vi "Check If User Data File is Empty.vi"(8 "error in (no error)":errorcluster, 11 "Refnum in":T1) -> (0 "error out":errorcluster, 3 "Refnum out":T1)   [LabVIEW 2018]
uses:
  <vilib>/Utility/config.llb/Config Data RefNum.ctl
  <vilib>/Utility/config.llb/Write Key (String).vi
  <vilib>/Utility/config.llb/NI_LVConfig.lvlib
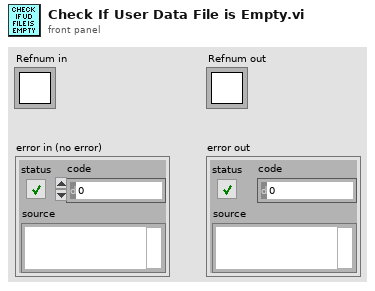
[diagram p1: front panel]
types:
  T1 = typedef "NI_LVConfig.lvlib/Config Data RefNum.ctl" = refnum<k1>
  T2 = enum16{"open", "replace", "create", "open or create", "replace or create", "replace or create with confirmation"}
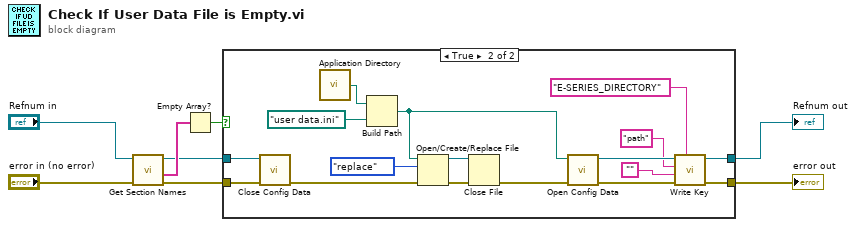
[diagram p0: block diagram]
diagram:
  n1 = call <vilib>:"Get Section Names.vi"("error in (no error)"="error in (no error)", "refnum"="Refnum in") -> ("error out"=w5:errorcluster, "section names"=w6:string[], "refnum out"=w3:T1)  [unwired: 7 in]
  n2 = Empty Array?(array=w6) -> (empty?=w4:bool)
  n3 = case shown="True" w4 {
    tunnel: w3 -> [w9 w22]
    tunnel: w5 -> [w10 w21]
    tunnel: [w10 w24] -> w8
    tunnel: [w9 w18] -> w1
    frame False {
    }
    frame True {
      n4 = call <vilib>:"Close Config Data.vi"("error in (no error)"=w21, "refnum"=w22) -> ("error out"=w17:errorcluster)  [unwired: 8 in, 1 out]
      n5 = call <vilib>:"Application Directory.vi"() -> ("Application Directory"=w20:path)
      n6 = Build Path(base path=w20, name or relative path=path "user data.ini") -> (appended path=w11:path)
      n7 = Open/Create/Replace File(file path (use dialog)=w11, error in=w17, operation (0:open)=T2."replace") -> (refnum out=w14:refnum<file>, error out=w15:errorcluster)  [unwired: 3 in, 1 out]
      n8 = Close File(refnum=w14, error in=w15) -> (error out=w13:errorcluster)  [unwired: 1 out]
      n9 = call <vilib>:"Open Config Data.vi"("error in (no error)"=w13, "configuration file path"=w11) -> ("error out"=w12:errorcluster, "refnum"=w27:T1)  [unwired: 7 in, 1 out]
      n10 = call-poly <vilib>:"Write Key.vi"("section"="E-SERIES_DIRECTORY", "error in (no error)"=w12, "value"="", "key"="path", "refnum"=w27) -> ("error out"=w24:errorcluster, "refnum out"=w18:T1)  [unwired: 4 in, 1 out]
    }
  }
  "error out" <- w8
  "Refnum out" <- w1
